vi "GV_Constructor.vi"(4 "Graph-ref":refnum<vi>, 5 "menu reference":refnum<k9>, 6 "StartupTagList":string[](array[string]), 7 "Pane":refnum<vi>, 8 "error in (no error)":errorcluster, 9 "Gserver-Queue":refnum<queue>, 10 "GviewName":string, 11 "Gviewer in":refnum<class "Gviewer.lvclass">) -> (0 "error out":errorcluster, 3 "Gviewer out":refnum<class "Gviewer.lvclass">)   [LabVIEW 2020, in "Sgraph_lib_V1.lvlib" / "Gviewer.lvclass"]
doc: "Constructor of the Sgraph Viewer : Set all default values, connect to Vserver, Setup default start conditions"
uses:
  Gviewer.lvclass
  Gserver/controls/Typedef_Gviewer-Query.ctl
  Gserver/controls/Typedef_QueryType.ctl
  <vilib>/Utility/miscctls.llb/LVPointTypeDef.ctl
  controls/ToolBarAppearance.ctl
  Gviewer.lvclass/Gviewer.ctl
  controls/Typedef_Gserver-Replies.ctl
  controls/Typedef_ServerActions.ctl
  FAMM/controls/Typedef_Gviewer_TagsUnits.ctl
  Common/controls/typedef_com_TagProp.ctl
  controls/Typedef_Live.ctl
  controls/Typedef_ZoomEvent.ctl
  controls/Typedef_SelProperties.ctl
  controls/Typedef_LineType.ctl
  Gserver/Gserver.lvclass
  Builds/Sgraph_lib_V1.lvlib
  FAMM/FAMM.lvclass
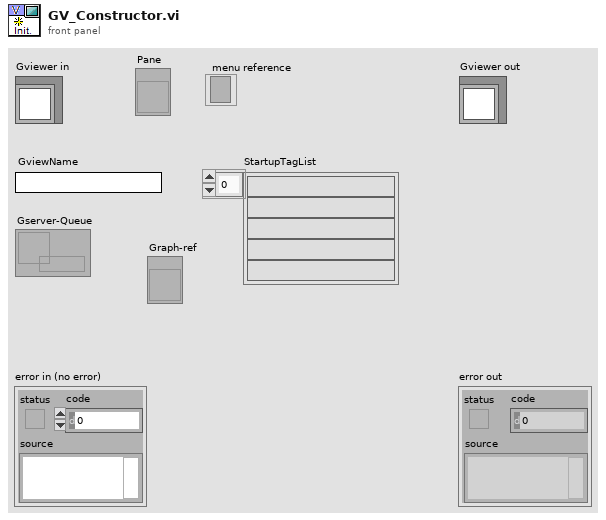
[diagram p1: front panel]
types:
  T1 = typedef "Sgraph_lib_V1.lvlib/Gviewer.lvclass/ToolBarAppearance.ctl" = enum16{"Bare", "Native", "Gradient"}
  T2 = typedef "LVPointTypeDef.ctl" = cluster{"Horizontal":i16, "Vertical":i16}
  T3 = typedef "Typedef_Gserver-Replies.ctl" = cluster{"ServerActions":T4, "data":variant, "Source":string, "Time Stamp":timestamp}
  T4 = typedef "Sgraph_lib_V1.lvlib/Typedef_ServerActions.ctl" = enum16{"GraphUpdate", "SendAllTags", "SendIniPath", "SetGeneralOptions", "EditTagsOpen", "EditTagsPresetSave", "EditTagsPresetLoad", "EditTagsClose", "NewTagSelection", "ExitGraph"}
  T5 = typedef "Sgraph_lib_V1.lvlib/Gserver.lvclass/Typedef_QueryType.ctl" = enum16{"Subscribe", "DataRequest", "RequestAllTags", "RequestIniPath", "FAMMstarted", "SetClientOptions", "GviewerUpdate", "OpenNewGraph", "CloseClient", "CloseAllClients", "Close Gserver", "OpenMemoryMap", "MeMapDataRequest", "MeMapDataResponse"}
  T6 = typedef "Sgraph_lib_V1.lvlib/Gserver.lvclass/Typedef_Gviewer-Query.ctl" = cluster{"Query_type":T5, "data":variant, "Source":string, "Time Stamp":timestamp}
  T7 = enum32{"Invalid", "Standard", "Closed", "Hidden", "Minimized", "Maximized"}
  T8 = typedef "Sgraph_lib_V1.lvlib/FAMM.lvclass/Typedef_Gviewer_TagsUnits.ctl" = cluster{"PAQ_TAGs":string[], "WAQ_TAGs":string[], "EAQ_TAGs":string[], "PAQtagProps":T9[], "WAQtagProps":T9[], "EAQtagProps":T9[]}
  T9 = typedef "Sgraph_lib_V1.lvlib/typedef_com_TagProp.ctl" = cluster{"Description":string, "EngUnits":string, "RangeH":dbl, "RangeL":dbl, "Resolution":i32, "Obsolete":bool, "ChangeDate":timestamp, "ChangeSource":string, "ChangeReason":string, "TagFunc":u32}
  T10 = typedef "Sgraph_lib_V1.lvlib/Gviewer.lvclass/Typedef_Live.ctl" = enum16{"Live View", "Freeze"}
  T11 = typedef "Typedef_ServerActions.ctl" = enum16{"GraphUpdate", "SendAllTags", "SendIniPath", "SetGeneralOptions", "EditTagsOpen", "EditTagsPresetSave", "EditTagsPresetLoad", "EditTagsClose", "NewTagSelection", "ExitGraph"}
  T12 = typedef "MenuStructure.ctl" = cluster{"After_tag":string, "MenuItems":T13[]}[]
  T13 = typedef "MenuItem.ctl" = cluster{"name":string, "tag":string, "checked":bool, "enabled":bool}
  T14 = typedef "Sgraph_lib_V1.lvlib/Gviewer.lvclass/Typedef_ZoomEvent.ctl" = cluster{"Time-Start":timestamp, "Time-End":timestamp, "TimeSpan(sec)":dbl, "Live":T10, "SelProperties":T15[], "Time Stamp":timestamp}
  T15 = typedef "Sgraph_lib_V1.lvlib/Gviewer.lvclass/Typedef_SelProperties.ctl" = cluster{"Color":u32, "LineType":T16, "max":dbl, "min":dbl}
  T16 = typedef "Sgraph_lib_V1.lvlib/Gviewer.lvclass/Typedef_LineType.ctl" = enum16{"num_bare", "num_MinMax_Area", "num_MinMax_Lines", "num_MinMax_Forfor", "num_Max_Area", "num_Max_Line", "num_Max_Forfor", "num_Min_Area", "num_Min_Line", "num_Min_Fosfor", "Boolean_Line_01", "Boolean_Area_01", "Boolean_Fosfor_01", "Boolean_Line_TF", "Boolean_Area_TF", "Boolean_Fosfor_TF", "Boolean_OnOff_Line", "Boolean_OnOff_Area", "Boolean_OnOff_Fosfor", "Boolean_spare", "StringEvent_Line", "StringEvent_TimeLine"}
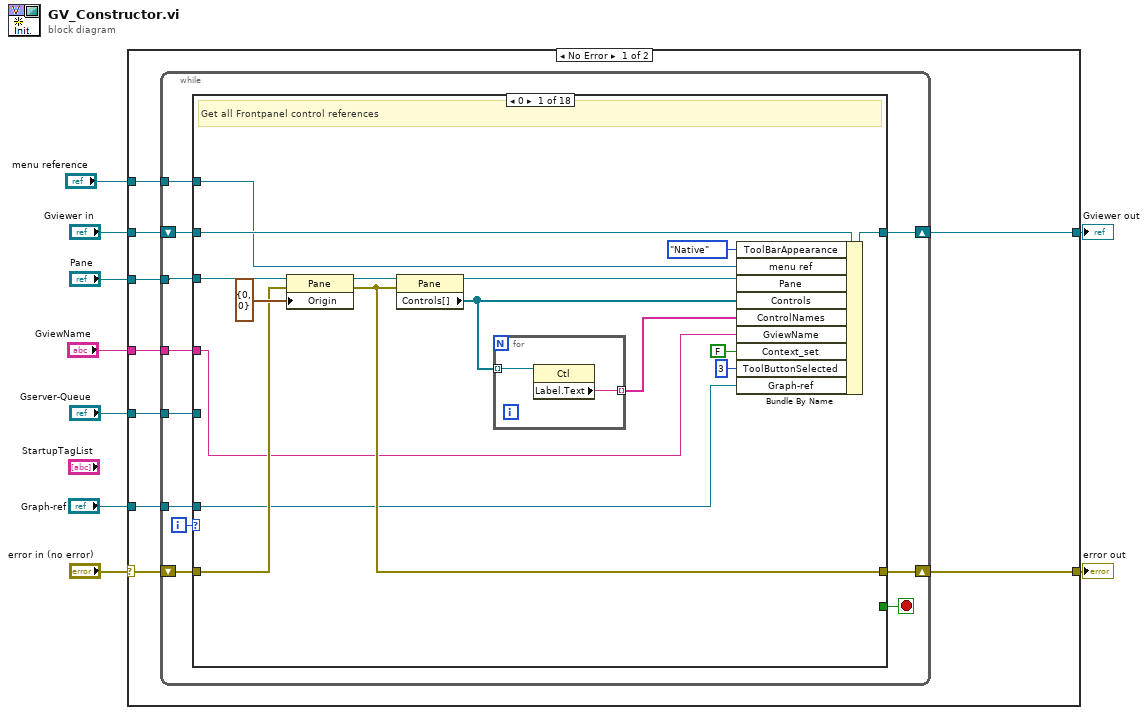
[diagram p0: block diagram]
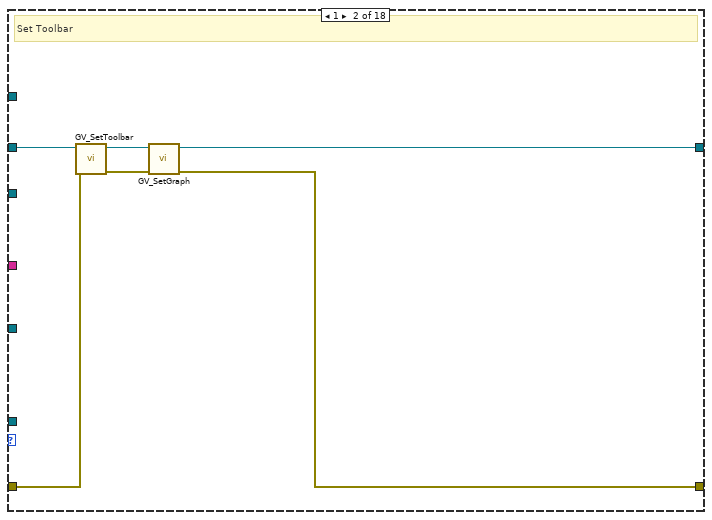
[diagram p2: hidden frame]
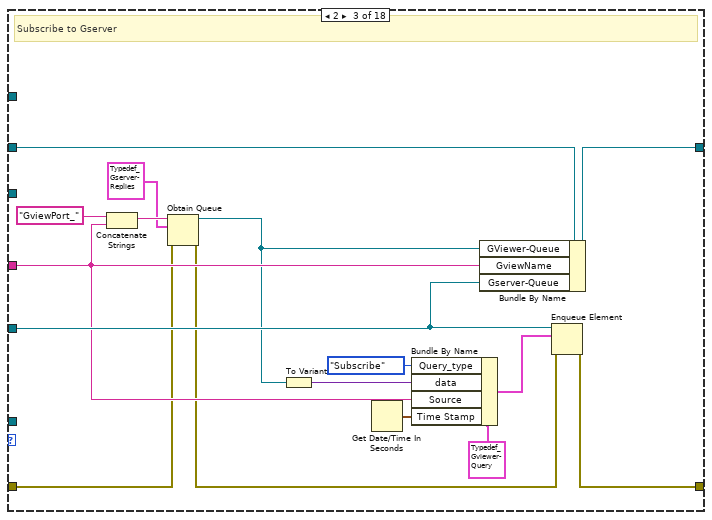
[diagram p3: hidden frame]
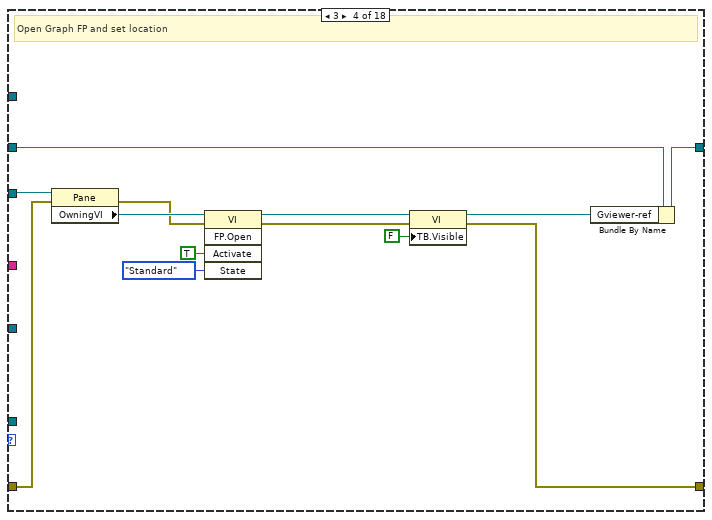
[diagram p4: hidden frame]
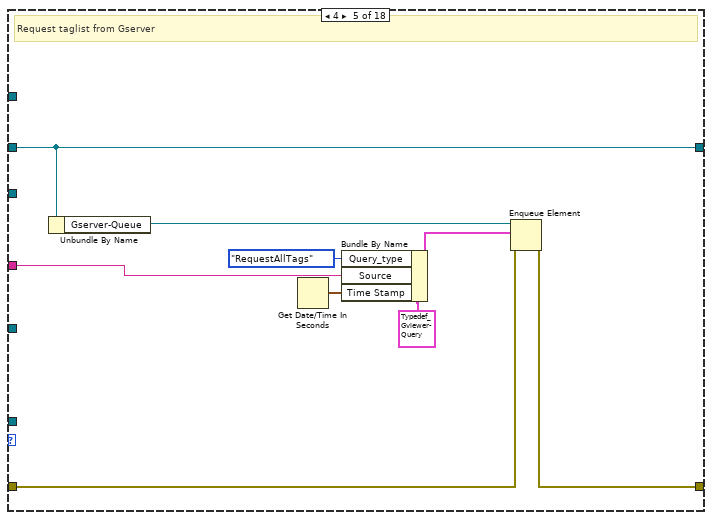
[diagram p5: hidden frame]
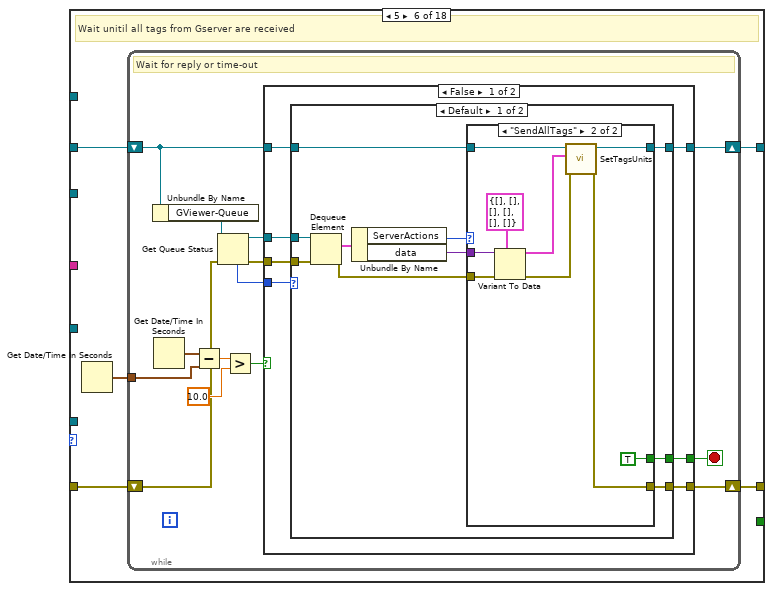
[diagram p6: hidden frame]
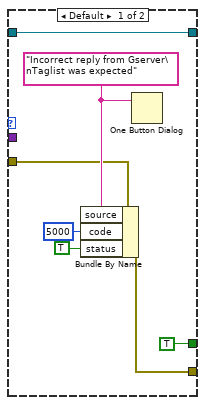
[diagram p7: hidden frame]
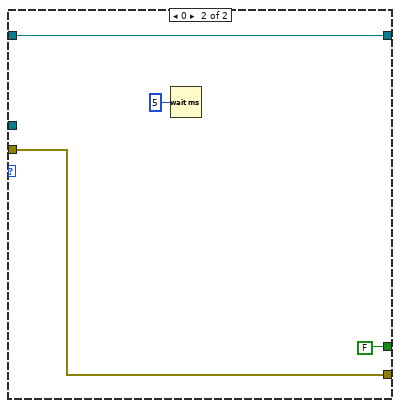
[diagram p8: hidden frame]
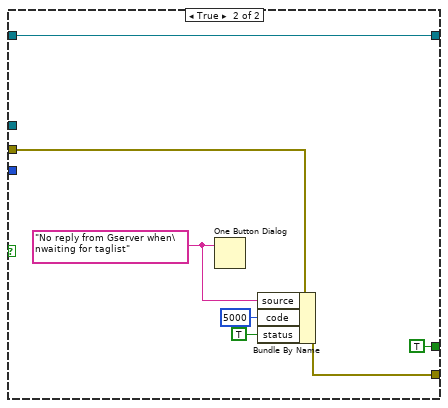
[diagram p9: hidden frame]
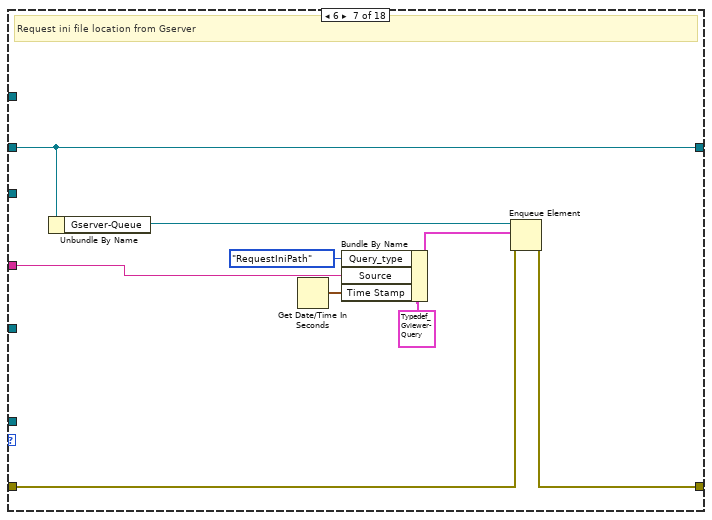
[diagram p10: hidden frame]
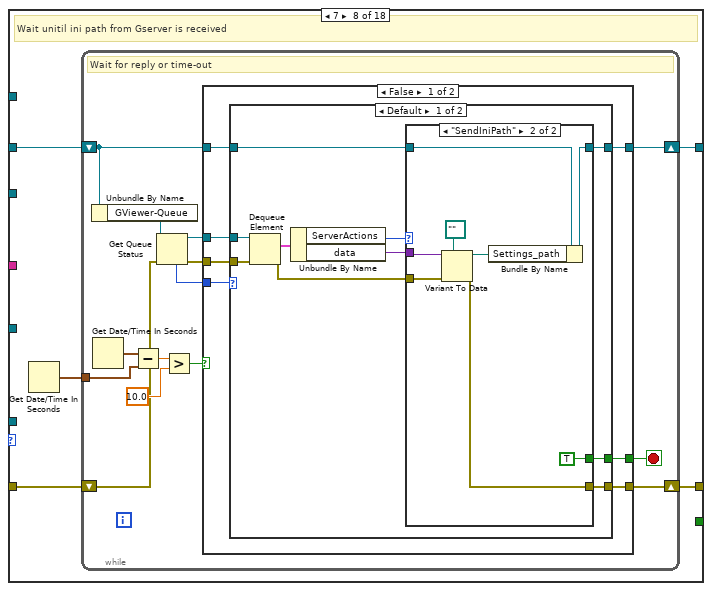
[diagram p11: hidden frame]
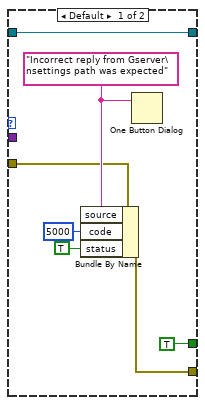
[diagram p12: hidden frame]
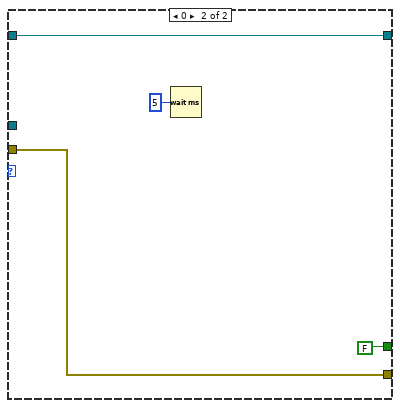
[diagram p13: hidden frame]
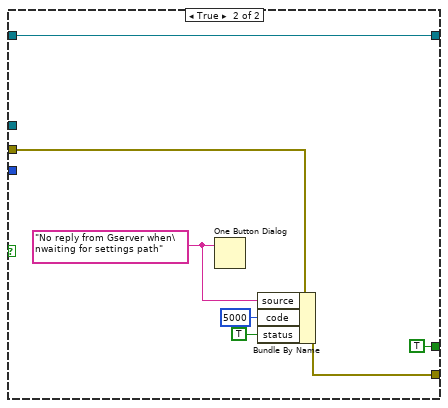
[diagram p14: hidden frame]
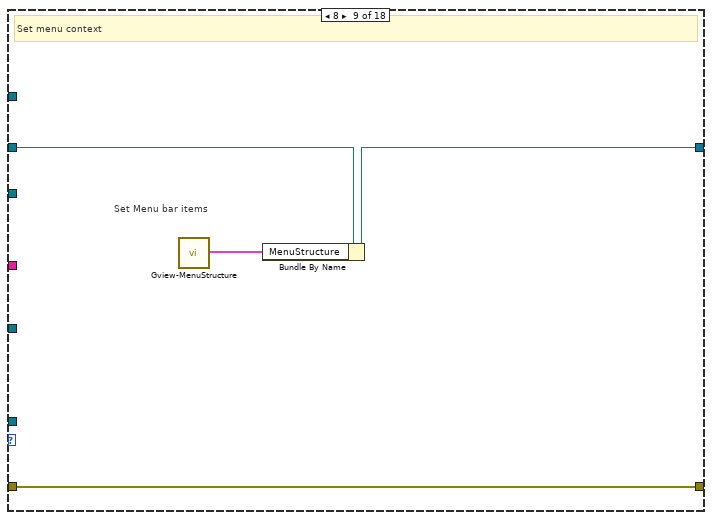
[diagram p15: hidden frame]
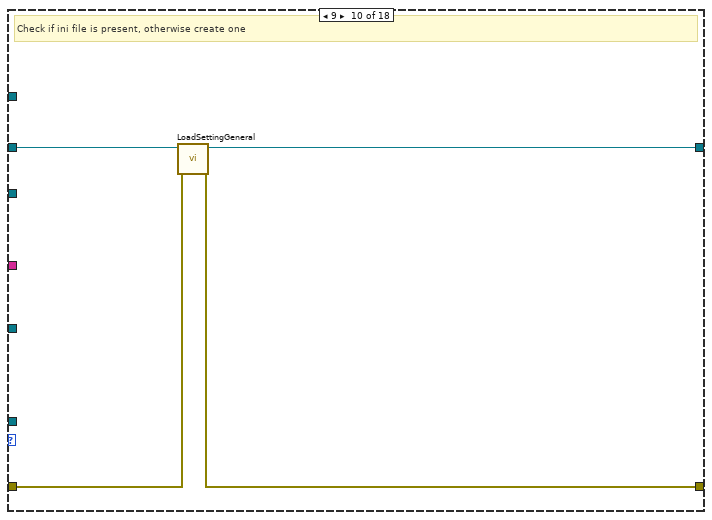
[diagram p16: hidden frame]
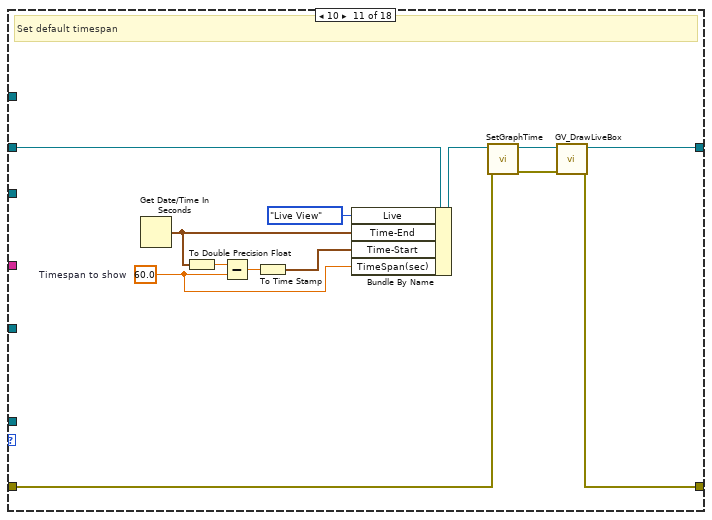
[diagram p17: hidden frame]
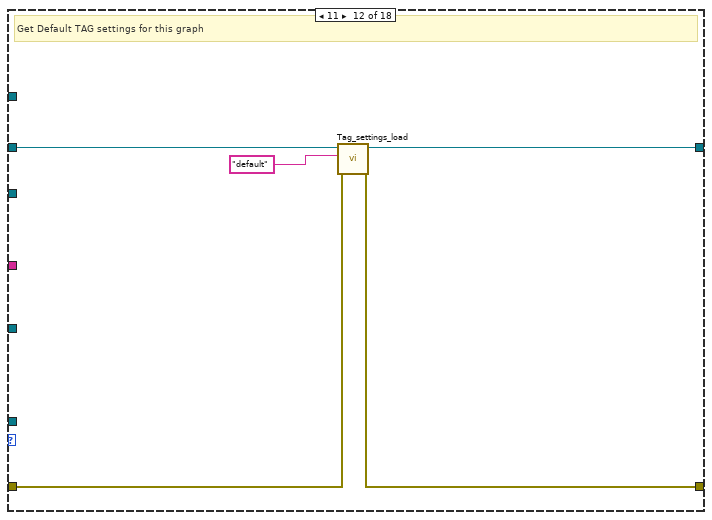
[diagram p18: hidden frame]
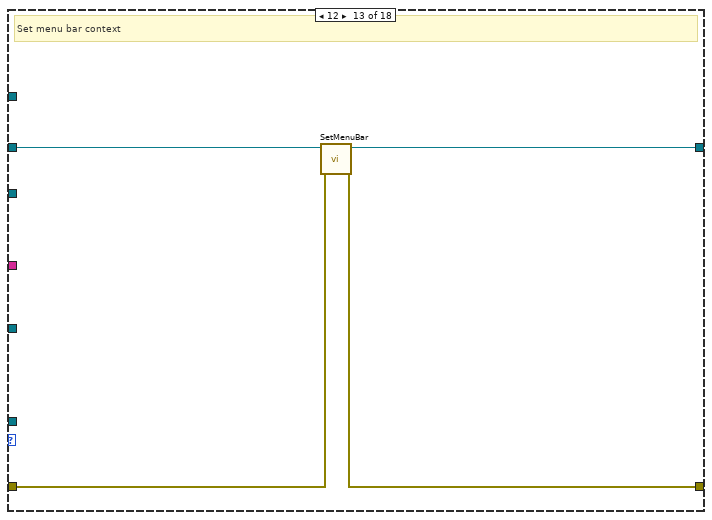
[diagram p19: hidden frame]
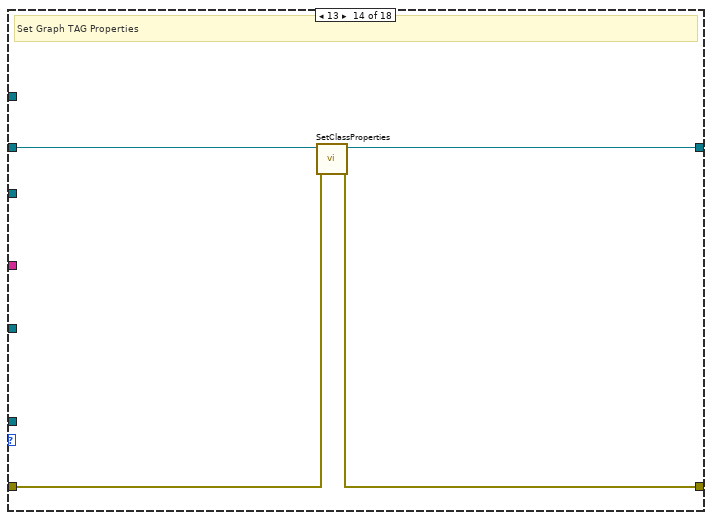
[diagram p20: hidden frame]
diagram:
  n1 = case shown="No Error" "error in (no error)" {
    selector: "error in (no error)" -> [w16 w294]
    tunnel: [w14 w294] -> w8
    tunnel: [w15 w293] -> w6
    tunnel: "Gviewer in" -> [w17 w293]
    tunnel: "Pane" -> [w18 _]
    tunnel: "GviewName" -> [w13 _]
    tunnel: "Gserver-Queue" -> [w12 _]
    tunnel: "menu reference" -> [w11 _]
    tunnel: "Graph-ref" -> [w10 _]
    frame No Error {
      n2 = while {
        tunnel: w18 -> [w25]
        shift-right: [w20] -> w15
        shift-left: w17 -> [w27]
        shift-right: [w28] -> w14
        shift-left: w16 -> [w19]
        tunnel: w13 -> [w24]
        tunnel: w12 -> [w23]
        tunnel: w11 -> [w22]
        tunnel: w10 -> [w21]
        i -> [w29]
        stop <- w26 stop-if-true
        n3 = case shown="0" w29 {
          tunnel: [w41 w48 w66 w72 w86 w92 w158 w164 w226 w230 w235 w248 w253 w256 w261 w267 w285 w291] -> w28
          tunnel: w27 -> [w40 w53 w68 w75 w91 w95 w163 w167 w229 w233 w246 w251 w254 w259 w262 w273 w283 w290]
          tunnel: [w39 w50 w69 w76 w91 w94 w163 w166 w227 w232 w236 w249 w255 w258 w263 w265 w288 w290] -> w20
          tunnel: [_ _ _ _ _ _ _ _ _ _ _ _ _ _ _ _ _ TRUE] -> w26
          tunnel: w25 -> [w45 _ _ w82 _ _ _ _ _ _ _ _ _ _ _ _ _ _]
          tunnel: w24 -> [w35 _ w60 _ w84 _ w156 _ _ _ _ _ _ _ _ _ _ _]
          tunnel: w23 -> [_ _ w67 _ _ _ _ _ _ _ _ _ _ _ _ _ _ _]
          tunnel: w22 -> [w34 _ _ _ _ _ _ _ _ _ _ _ _ _ _ _ _ _]
          tunnel: w21 -> [w30 _ _ _ _ _ _ _ _ _ _ _ _ _ _ _ _ _]
          tunnel: w19 -> [w43 w52 w57 w81 w85 w93 w157 w165 w226 w231 w239 w247 w252 w257 w260 w269 w286 w291]
          frame 0 {
            # "Get all Frontpanel control references"
            n4 = property class="Pane"(reference=w45, error in=w43, "Origin"=T2 {"Horizontal"=0, "Vertical"=0}) -> (reference out=w42:refnum<vi>, error out=w41:errorcluster)
            n5 = property class="Pane"(reference=w42, error in=w41) -> (reference out=w36:refnum<vi>, "Controls[]"=w38:refnum<vi>[])  [unwired: 1 out]
            n6 = for {
              tunnel: w38 -> [w47] mode=indexing
              tunnel: [w46] -> w37 mode=indexing
              n7 = property class="Ctl"(reference=w47) -> ("Label.Text"=w46:string)  [unwired: 1 in, 2 out]
            }
            n8 = Bundle By Name(cluster=w40, "ToolBarAppearance"=ToolBarAppearance."Native", "menu ref"=w34, "Pane"=w36, "Controls"=w38, "ControlNames"=w37, "GviewName"=w35, "Context_set"=FALSE, "ToolButtonSelected"=3, "Graph-ref"=w30) -> (w39:refnum<class "Gviewer.lvclass">)
          }
          frame 1 {
            # "Set Toolbar"
            n9 = call "GV_SetToolbar.vi"("error in (no error)"=w52, "Gviewer in"=w53) -> ("error out"=w49:errorcluster, "Gviewer out"=w51:refnum<class "Gviewer.lvclass">)  [unwired: 8 in]
            n10 = call "GV_SetGraph.vi"("error in (no error)"=w49, "Gviewer in"=w51) -> ("error out"=w48:errorcluster, "Gviewer out"=w50:refnum<class "Gviewer.lvclass">)  [unwired: 8 in]
          }
          frame 2 {
            # "Subscribe to Gserver"
            n11 = Concatenate Strings("GviewPort_", w60) -> (w59:string)
            n12 = Obtain Queue(name (unnamed)=w59, element data type=T3 {"ServerActions"=enum."GraphUpdate", "data"=variant, "Source"="", "Time Stamp"=timestamp(0 s since 1904-01-01)} ("Query"), error in (no error)=w57) -> (queue out=w54:refnum<queue>, error out=w58:errorcluster)  [unwired: 2 in, 1 out]
            n13 = To Variant(anything=w54) -> (Variant=w55:variant)
            n14 = Get Date/Time In Seconds() -> (seconds since 1Jan1904=w62:timestamp)
            n15 = Bundle By Name(cluster=T6 {"Query_type"=enum."Subscribe", "data"=variant, "Source"="", "Time Stamp"=timestamp(0 s since 1904-01-01)} ("element"), "Query_type"=Typedef_QueryType."Subscribe", "data"=w55, "Source"=w60, "Time Stamp"=w62) -> (w64:T6)
            n16 = Bundle By Name(cluster=w68, "GViewer-Queue"=w54, "GviewName"=w60, "Gserver-Queue"=w67) -> (w69:refnum<class "Gviewer.lvclass">)
            n17 = Enqueue Element(queue=w67, element=w64, error in (no error)=w58) -> (error out=w66:errorcluster)  [unwired: 1 in, 2 out]
          }
          frame 3 {
            # "Open Graph FP and set location"
            n18 = property class="Pane"(reference=w82, error in=w81) -> (error out=w79:errorcluster, "OwningVI"=w80:refnum<vi>)  [unwired: 1 out]
            n19 = invoke class="VI" method="FP.Open"(reference=w80, error in=w79, "Activate"=TRUE ("Activate?"), "State"=T7."Standard") -> (reference out=w71:refnum<vi>, error out=w70:errorcluster)  [unwired: 1 in, 3 out]
            n20 = property class="VI"(reference=w71, error in=w70, "TB.Visible"=FALSE ("Tool Bar:Visible")) -> (reference out=w73:refnum<vi>, error out=w72:errorcluster)
            n21 = Bundle By Name(cluster=w75, "Gviewer-ref"=w73) -> (w76:refnum<class "Gviewer.lvclass">)
          }
          frame 4 {
            # "Request taglist from Gserver"
            n22 = Unbundle By Name(w91) -> ("Gserver-Queue"=w88:refnum<queue>)
            n23 = Get Date/Time In Seconds() -> (seconds since 1Jan1904=w83:timestamp)
            n24 = Bundle By Name(cluster=T6 {"Query_type"=enum."Subscribe", "data"=variant, "Source"="", "Time Stamp"=timestamp(0 s since 1904-01-01)} ("element"), "Query_type"=Typedef_QueryType."RequestAllTags", "Source"=w84, "Time Stamp"=w83) -> (w87:T6)
            n25 = Enqueue Element(queue=w88, element=w87, error in (no error)=w85) -> (error out=w86:errorcluster)  [unwired: 1 in, 2 out]
          }
          frame 5 {
            # "Wait unitil all tags from Gserver are received"
            n26 = Get Date/Time In Seconds() -> (seconds since 1Jan1904=w96:timestamp)
            n27 = while {
              tunnel: w96 -> [w109]
              shift-right: [w105] -> w94
              shift-left: w95 -> [w102]
              shift-right: [w104] -> w92
              shift-left: w93 -> [w98]
              stop <- w103 stop-if-true
              # "Wait for reply or time-out"
              n28 = Unbundle By Name(w102) -> ("GViewer-Queue"=w101:refnum<queue>)
              n29 = Get Date/Time In Seconds() -> (seconds since 1Jan1904=w110:timestamp)
              n30 = Subtract(x=w110, y=w109) -> (x-y=w108:dbl)
              n31 = Get Queue Status(queue=w101, error in (no error)=w98) -> (queue out=w100:refnum<queue>, error out=w97:errorcluster, # elements in queue=w99:i32)  [unwired: 1 in, 5 out]
              n32 = Greater?(x=w108, y=10.0) -> (0:w106:bool)
              n33 = case shown="False" w106 {
                tunnel: w102 -> [w116 w154]
                tunnel: [w115 w154] -> w105
                tunnel: [w114 w150] -> w104
                tunnel: [w111 TRUE] -> w103
                tunnel: w100 -> [w113 _]
                tunnel: w99 -> [w117 _]
                tunnel: w97 -> [w112 w149]
                frame False {
                  n34 = case shown="Default" w117 {
                    tunnel: w116 -> [w123 w147]
                    tunnel: [w122 w147] -> w115
                    tunnel: [w121 w145] -> w114
                    tunnel: w113 -> [w126 _]
                    tunnel: w112 -> [w125 w145]
                    tunnel: [w119 FALSE] -> w111
                    frame Default {
                      n35 = Dequeue Element(queue=w126, error in (no error)=w125) -> (element=w127:T3, error out=w120:errorcluster)  [unwired: 1 in, 2 out]
                      n36 = Unbundle By Name(w127) -> ("ServerActions"=w124:T11, "data"=w118:variant)
                      n37 = case shown="\"SendAllTags\"" w124 {
                        tunnel: w123 -> [w134 w139]
                        tunnel: [w134 w138] -> w122
                        tunnel: [w129 w135] -> w121
                        tunnel: w120 -> [w128 w141]
                        tunnel: [TRUE TRUE] -> w119
                        tunnel: w118 -> [_ w142]
                        frame Default {
                          w130 = "Incorrect reply from Gserver\nTaglist was expected" ("message")
                          n38 = Bundle By Name(cluster=w128, "source"=w130, "code"=5000, "status"=TRUE) -> (w129:errorcluster)
                          n39 = One Button Dialog(message=w130) -> ()  [unwired: 1 in, 1 out]
                        }
                        frame "SendAllTags" {
                          n40 = Variant To Data(error in=w141, type=T8 {"PAQ_TAGs"=[], "WAQ_TAGs"=[], "EAQ_TAGs"=[], "PAQtagProps"=[], "WAQtagProps"=[], "EAQtagProps"=[]} ("Tags_Units"), Variant=w142) -> (data=w137:T8, error out=w136:errorcluster)
                          n41 = call "SetTagsUnits.vi"("error in (no error)"=w136, "Tags_Units"=w137, "Gviewer in"=w139) -> ("error out"=w135:errorcluster, "Gviewer out"=w138:refnum<class "Gviewer.lvclass">)  [unwired: 7 in]
                        }
                      }
                    }
                    frame 0 {
                      n42 = Wait (ms)(milliseconds to wait=u32 5) -> ()  [unwired: 1 out]
                    }
                  }
                }
                frame True {
                  w148 = "No reply from Gserver when\nwaiting for taglist" ("message")
                  n43 = One Button Dialog(message=w148) -> ()  [unwired: 1 in, 1 out]
                  n44 = Bundle By Name(cluster=w149, "source"=w148, "code"=5000, "status"=TRUE) -> (w150:errorcluster)
                }
              }
            }
          }
          frame 6 {
            # "Request ini file location from Gserver"
            n45 = Unbundle By Name(w163) -> ("Gserver-Queue"=w160:refnum<queue>)
            n46 = Get Date/Time In Seconds() -> (seconds since 1Jan1904=w155:timestamp)
            n47 = Bundle By Name(cluster=T6 {"Query_type"=enum."Subscribe", "data"=variant, "Source"="", "Time Stamp"=timestamp(0 s since 1904-01-01)} ("element"), "Query_type"=Typedef_QueryType."RequestIniPath", "Source"=w156, "Time Stamp"=w155) -> (w159:T6)
            n48 = Enqueue Element(queue=w160, element=w159, error in (no error)=w157) -> (error out=w158:errorcluster)  [unwired: 1 in, 2 out]
          }
          frame 7 {
            # "Wait unitil ini path from Gserver is received"
            n49 = Get Date/Time In Seconds() -> (seconds since 1Jan1904=w168:timestamp)
            n50 = while {
              tunnel: w168 -> [w181]
              shift-right: [w177] -> w166
              shift-left: w167 -> [w174]
              shift-right: [w176] -> w164
              shift-left: w165 -> [w170]
              stop <- w175 stop-if-true
              # "Wait for reply or time-out"
              n51 = Unbundle By Name(w174) -> ("GViewer-Queue"=w173:refnum<queue>)
              n52 = Get Date/Time In Seconds() -> (seconds since 1Jan1904=w182:timestamp)
              n53 = Subtract(x=w182, y=w181) -> (x-y=w180:dbl)
              n54 = Get Queue Status(queue=w173, error in (no error)=w170) -> (queue out=w172:refnum<queue>, error out=w169:errorcluster, # elements in queue=w171:i32)  [unwired: 1 in, 5 out]
              n55 = Greater?(x=w180, y=10.0) -> (0:w178:bool)
              n56 = case shown="False" w178 {
                tunnel: w174 -> [w188 w225]
                tunnel: [w187 w225] -> w177
                tunnel: [w186 w221] -> w176
                tunnel: [w183 TRUE] -> w175
                tunnel: w172 -> [w185 _]
                tunnel: w171 -> [w189 _]
                tunnel: w169 -> [w184 w220]
                frame False {
                  n57 = case shown="Default" w189 {
                    tunnel: w188 -> [w195 w218]
                    tunnel: [w194 w218] -> w187
                    tunnel: [w193 w216] -> w186
                    tunnel: w185 -> [w198 _]
                    tunnel: w184 -> [w197 w216]
                    tunnel: [w191 FALSE] -> w183
                    frame Default {
                      n58 = Dequeue Element(queue=w198, error in (no error)=w197) -> (element=w199:T3, error out=w192:errorcluster)  [unwired: 1 in, 2 out]
                      n59 = Unbundle By Name(w199) -> ("ServerActions"=w196:T11, "data"=w190:variant)
                      n60 = case shown="\"SendIniPath\"" w196 {
                        tunnel: w195 -> [w206 w212]
                        tunnel: [w206 w211] -> w194
                        tunnel: [w201 w209] -> w193
                        tunnel: w192 -> [w200 w208]
                        tunnel: [TRUE TRUE] -> w191
                        tunnel: w190 -> [_ w210]
                        frame Default {
                          w202 = "Incorrect reply from Gserver\nsettings path was expected" ("message")
                          n61 = Bundle By Name(cluster=w200, "source"=w202, "code"=5000, "status"=TRUE) -> (w201:errorcluster)
                          n62 = One Button Dialog(message=w202) -> ()  [unwired: 1 in, 1 out]
                        }
                        frame "SendIniPath" {
                          n63 = Variant To Data(error in=w208, type=path "" ("Path"), Variant=w210) -> (data=w213:path, error out=w209:errorcluster)
                          n64 = Bundle By Name(cluster=w212, "Settings_path"=w213) -> (w211:refnum<class "Gviewer.lvclass">)
                        }
                      }
                    }
                    frame 0 {
                      n65 = Wait (ms)(milliseconds to wait=u32 5) -> ()  [unwired: 1 out]
                    }
                  }
                }
                frame True {
                  w219 = "No reply from Gserver when\nwaiting for settings path" ("message")
                  n66 = One Button Dialog(message=w219) -> ()  [unwired: 1 in, 1 out]
                  n67 = Bundle By Name(cluster=w220, "source"=w219, "code"=5000, "status"=TRUE) -> (w221:errorcluster)
                }
              }
            }
          }
          frame 8 {
            # "Set Menu bar items"
            # "Set menu context"
            n68 = call "Gview-MenuStructure.vi"() -> ("MenuStructure"=w228:T12)  [unwired: 2 in]
            n69 = Bundle By Name(cluster=w229, "MenuStructure"=w228) -> (w227:refnum<class "Gviewer.lvclass">)
          }
          frame 9 {
            # "Check if ini file is present, otherwise create one"
            n70 = call "LoadSettingGeneral.vi"("error in (no error)"=w231, "Gviewer in"=w233) -> ("error out"=w230:errorcluster, "Gviewer out"=w232:refnum<class "Gviewer.lvclass">)  [unwired: 7 in, 1 out]
          }
          frame 10 {
            w241 = 60.0  # Timespan to show
            # "Set default timespan"
            n71 = Get Date/Time In Seconds() -> (seconds since 1Jan1904=w245:timestamp)
            n72 = To Double Precision Float(number=w245) -> (double precision float=w244:dbl)
            n73 = Subtract(x=w244, y=w241) -> (x-y=w243:dbl)
            n74 = To Time Stamp(1:w243) -> (0:w242:timestamp)
            n75 = Bundle By Name(cluster=w246, "Live"=Typedef_Live."Live View", "Time-End"=w245, "Time-Start"=w242, "TimeSpan(sec)"=w241) -> (w240:refnum<class "Gviewer.lvclass">)
            n76 = call "SetGraphTime.vi"("error in (no error)"=w239, "Gviewer in"=w240) -> ("error out"=w237:errorcluster, "Gviewer out"=w238:refnum<class "Gviewer.lvclass">)  [unwired: 8 in]
            n77 = call "GV_DrawLiveBox.vi"("error in (no error)"=w237, "Gviewer in"=w238) -> ("error out"=w235:errorcluster, "Gviewer out"=w236:refnum<class "Gviewer.lvclass">)  [unwired: 8 in]
          }
          frame 11 {
            # "Get Default TAG settings for this graph"
            n78 = call "Tag_settings_load.vi"("error in (no error)"=w247, "PresetName"="default" ("SettingsName"), "Gviewer in"=w251) -> ("error out"=w248:errorcluster, "Gviewer out"=w249:refnum<class "Gviewer.lvclass">)  [unwired: 7 in]
          }
          frame 12 {
            # "Set menu bar context"
            n79 = call "SetMenuBar.vi"("error in (no error)"=w252, "Gviewer in"=w254) -> ("error out"=w253:errorcluster, "Gviewer out"=w255:refnum<class "Gviewer.lvclass">)  [unwired: 8 in]
          }
          frame 13 {
            # "Set Graph TAG Properties"
            n80 = call "SetClassProperties.vi"("error in (no error)"=w257, "Gviewer in"=w259) -> ("error out"=w256:errorcluster, "Gviewer out"=w258:refnum<class "Gviewer.lvclass">)  [unwired: 8 in]
          }
          frame 14 {
            # "Request first frame from Gserver"
            n81 = call "Request_Gserver_Update.vi"("error in (no error)"=w260, "Gviewer in"=w262) -> ("error out"=w261:errorcluster, "Gviewer out"=w263:refnum<class "Gviewer.lvclass">)  [unwired: 8 in]
          }
          frame 15 {
            # "Determine if Legend is visible at startup"
            n82 = call "GV_LegendOnOff.vi"("error in (no error)"=w269, "On?"=FALSE, "Gviewer in"=w273) -> ("error out"=w270:errorcluster, "Visible?"=w271:bool, "Gviewer out"=w272:refnum<class "Gviewer.lvclass">)  [unwired: 6 in]
            n83 = call "SetMenuTagChecked.vi"("error in (no error)"=w270, "Checked"=w271, "TAG"="Legend", "Gviewer in"=w272) -> ("error out"=w275:errorcluster, "Gviewer out"=w276:refnum<class "Gviewer.lvclass">)  [unwired: 6 in]
            n84 = call "SetMenuBar.vi"("error in (no error)"=w275, "Gviewer in"=w276) -> ("error out"=w267:errorcluster, "Gviewer out"=w266:refnum<class "Gviewer.lvclass">)  [unwired: 8 in]
            n85 = Bundle By Name(cluster=w266, "PlotSelected"=-1) -> (w265:refnum<class "Gviewer.lvclass">)
          }
          frame 16 {
            w284 = T14 {"Time-Start"=timestamp(0 s since 1904-01-01), "Time-End"=timestamp(0 s since 1904-01-01), "TimeSpan(sec)"=0.0, "Live"=enum."Live View", "SelProperties"=[], "Time Stamp"=timestamp(0 s since 1904-01-01)} ("ZoomEvent")
            # "Add first default setting to undo memory"
            n86 = Unbundle By Name(w283) -> ("Time-Start"=w282:timestamp, "Time-End"=w281:timestamp, "TimeSpan(sec)"=w280:dbl, "Live"=w278:T10, "SelProperties"=w279:T15[])
            n87 = Get Date/Time In Seconds() -> (seconds since 1Jan1904=w277:timestamp)
            n88 = Bundle By Name(cluster=w284, "Time-Start"=w282, "Time-End"=w281, "TimeSpan(sec)"=w280, "Live"=w278, "SelProperties"=w279, "Time Stamp"=w277) -> ()  [unwired: 1 out]
            n89 = call "GV_Undo_add.vi"("error in (no error)"=w286, "ZoomEvent"=w284, "Gviewer in"=w283) -> ("error out"=w285:errorcluster, "Gviewer out"=w287:refnum<class "Gviewer.lvclass">)  [unwired: 7 in]
            n90 = Bundle By Name(cluster=w287, "MaxUndoDepth"=20) -> (w288:refnum<class "Gviewer.lvclass">)
          }
          frame Default {
            # "Last init frame"
          }
        }
      }
    }
    frame Error {
    }
  }
  "error out" <- w8
  "Gviewer out" <- w6
